vi "DAQ Judge.vi"(10 "Time and Data In":T3, 11 "Sample Settings":T1={"设备信息"={"初始索引子集"=[], "模拟信号采集通道"="Dev1", "数字-供电"="", "数字-光控"="", "光控设备"="", "光电设备分离？"=FALSE, "光谱保存路径"=path "", "环数"=0}, "测量控制"={"测头拿起"=FALSE, "起始保存"=FALSE, "测头供电"=TRUE, "测头出光"=TRUE}, "测量"={"每波长测量次数"=5, "波长"=[0, 0, 0, 0, 0, 0], "起始周期"=0, "起始测量周期"=0}, "等待"={"等待时间(s)"=0.0, "等待方式"=FALSE, "每x周期/点等待"=8, "等待时"=enum."无电无光"}, "校准"={"暗电流校准值初值"=[], "温度校准值"=[0.0, 0.0, 0.0, 0.0, 0.0, 0.0, 0.00013, 0.00013, 0.00013, 0.00013, 0.00013, 0.00013], "校准模式"=enum."逐周期"}, "图表相关"={"文件-时间"=""}, "CSM"={"CSM Name"=""}}) -> (1 "等待？":bool, 2 "Time and Data Out":T3)   [LabVIEW 2026, in "UI-无创.lvlib" / "Acquisition.lvlib"]
uses:
  Acquisition.lvlib
  Supports/Time and Data_OP.ctl
  Supports/Sample Settings.ctl
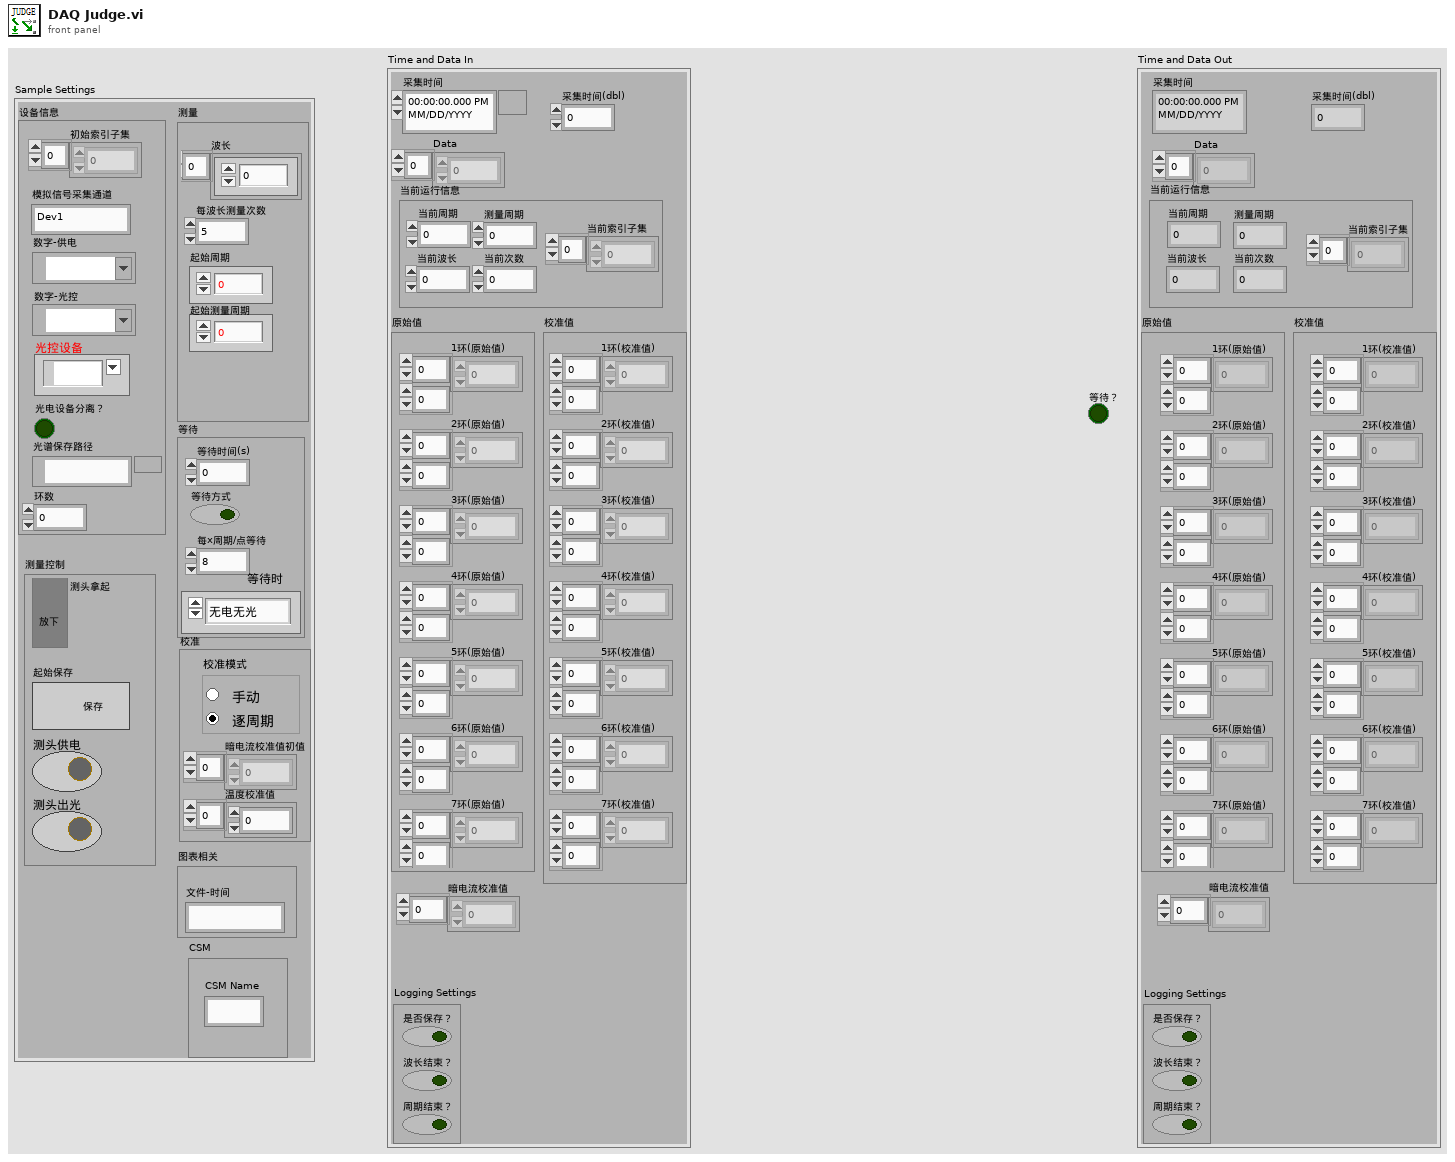
[diagram p1: front panel]
types:
  T1 = typedef "UI-无创.lvlib/Sample Settings.ctl" = cluster{"设备信息":cluster{"初始索引子集":i8[], "模拟信号采集通道":string, "数字-供电":refnum<k21>, "数字-光控":refnum<k21>, "光控设备":tag, "光电设备分离？":bool, "光谱保存路径":path, "环数":u8}, "测量控制":cluster{"测头拿起":bool, "起始保存":bool, "测头供电":bool, "测头出光":bool}, "测量":cluster{"每波长测量次数":i32, "波长":i32[], "起始周期":i32, "起始测量周期":i32}, "等待":cluster{"等待时间(s)":dbl, "等待方式":bool, "每x周期/点等待":i32, "等待时":enum16{"无电无光", "有电无光", "无电有光", "有电有光"}}, "校准":cluster{"暗电流校准值初值":dbl[], "温度校准值":dbl[], "校准模式":T2}, "图表相关":cluster{"文件-时间":string}, "CSM":cluster{"CSM Name":string}}
  T2 = typedef "UI-无创.lvlib/暗电流校准模式.ctl" = enum32{"手动", "逐周期"}
  T3 = typedef "UI-无创.lvlib/Time and Data_OP.ctl" = cluster{"采集时间":timestamp, "采集时间(dbl)":dbl, "Data":dbl[], "当前运行信息":cluster{"当前周期":i32, "当前次数":i32, "测量周期":i32, "当前索引子集":i8[], "当前波长":i32}, "暗电流校准值":dbl[], "Logging Settings":cluster{"是否保存？":bool, "波长结束？":bool, "周期结束？":bool}, "原始值":cluster{"1环(原始值)":dbl[][], "2环(原始值)":dbl[][], "3环(原始值)":dbl[][], "4环(原始值)":dbl[][], "5环(原始值)":dbl[][], "6环(原始值)":dbl[][], "7环(原始值)":dbl[][]}, "校准值":cluster{"1环(校准值)":dbl[][], "2环(校准值)":dbl[][], "3环(校准值)":dbl[][], "4环(校准值)":dbl[][], "5环(校准值)":dbl[][], "6环(校准值)":dbl[][], "7环(校准值)":dbl[][]}}
  T4 = cluster{"Time and Data In":T3, "Sample Settings":T1}
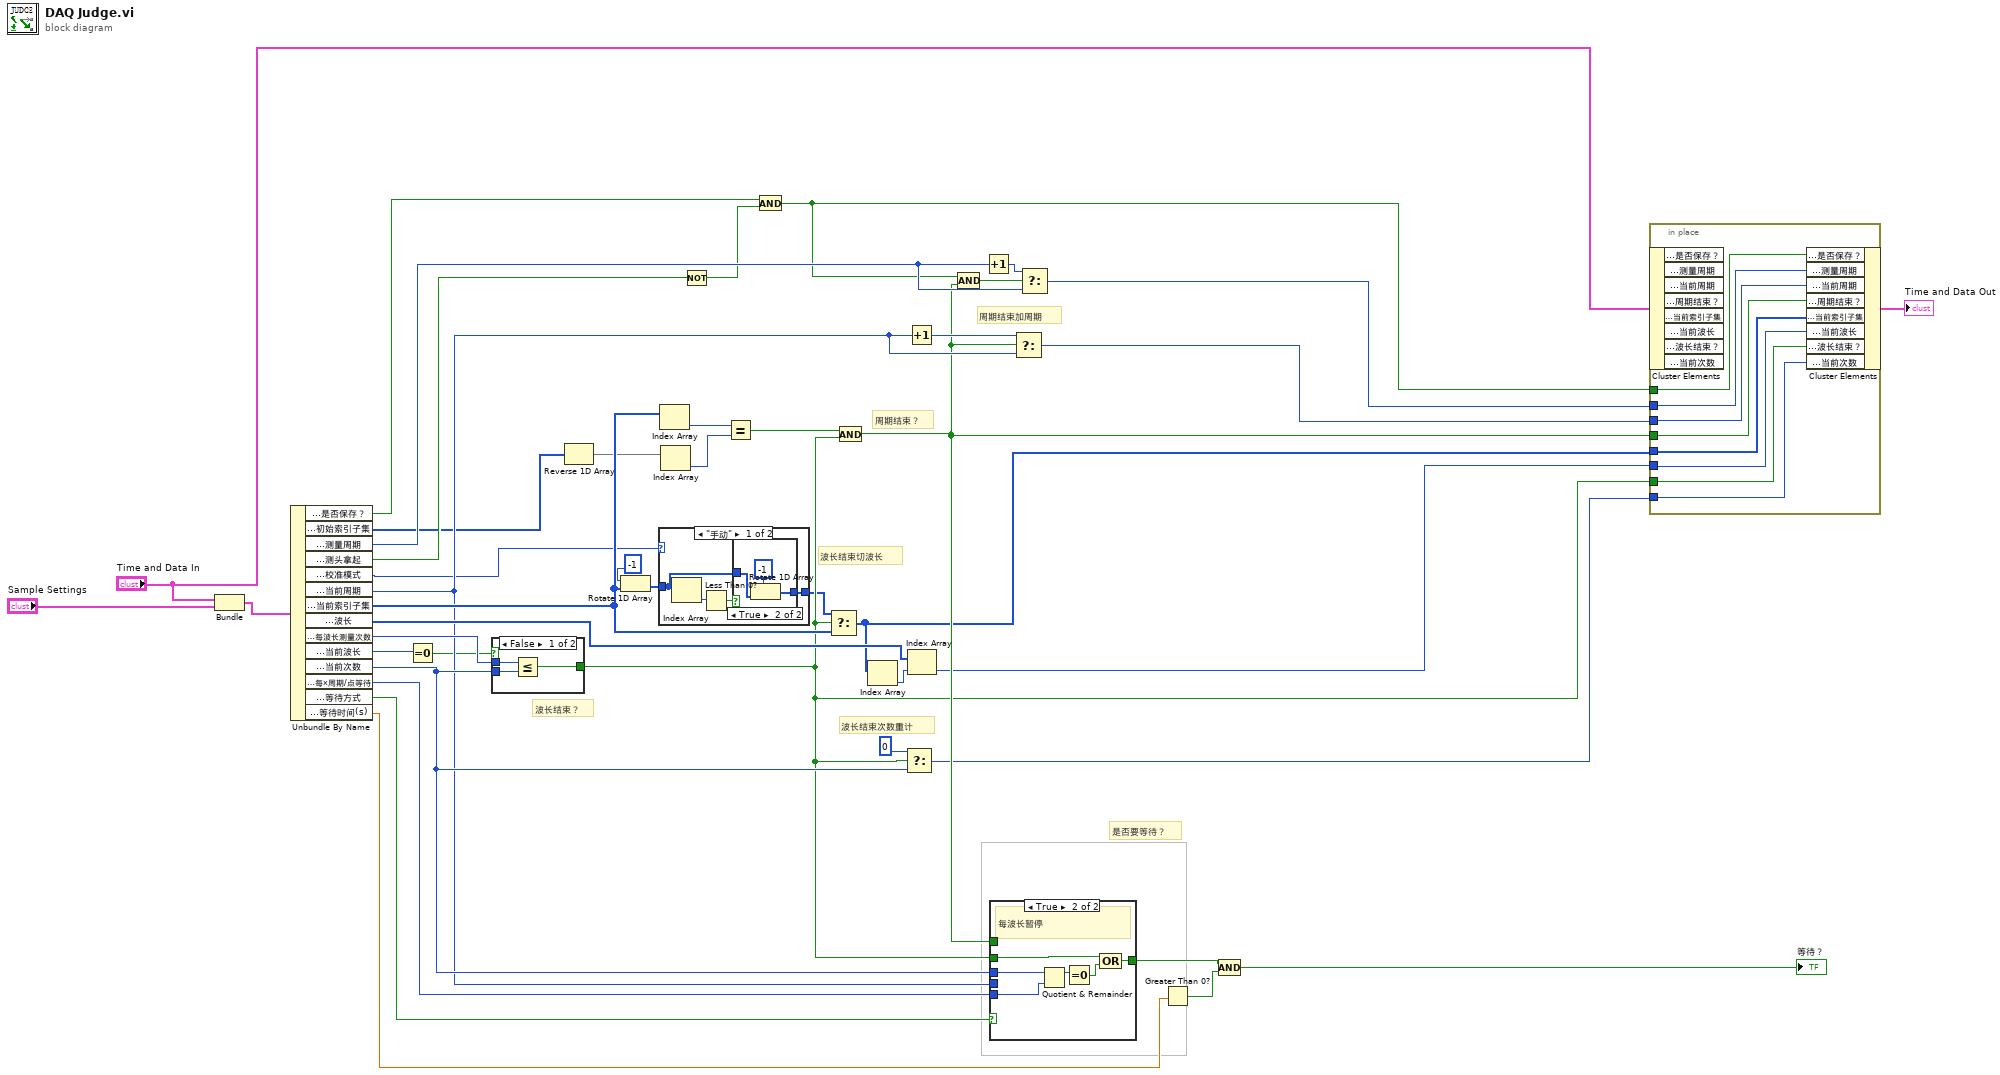
[diagram p0: block diagram]
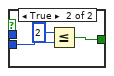
[diagram p4: hidden frame]
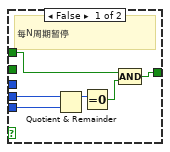
[diagram p5: hidden frame]
diagram:
  # "波长结束？"
  # "波长结束次数重计"
  # "波长结束切波长"
  # "是否要等待？"
  # "周期结束？"
  # "周期结束加周期"
  n1 = Bundle("Time and Data In"="Time and Data In", "Sample Settings"="Sample Settings") -> (w28:T4)  [unwired: 1 in]
  n2 = Unbundle By Name(w28) -> ("Time and Data In.Logging Settings.是否保存？"=w23:bool, "Sample Settings.设备信息.初始索引子集"=w7:i8[], "Time and Data In.当前运行信息.测量周期"=w30:i32, "Sample Settings.测量控制.测头拿起"=w22:bool, "Sample Settings.校准.校准模式"=w3:T2, "Time and Data In.当前运行信息.当前周期"=w33:i32, "Time and Data In.当前运行信息.当前索引子集"=w39:i8[], "Sample Settings.测量.波长"=w38:i32[], "Sample Settings.测量.每波长测量次数"=w41:i32, "Time and Data In.当前运行信息.当前波长"=w6:i32, "Time and Data In.当前运行信息.当前次数"=w34:i32, "Sample Settings.等待.每x周期/点等待"=w27:i32, "Sample Settings.等待.等待方式"=w26:bool, "Sample Settings.等待.等待时间(s)"=w20:dbl)
  n3 = Equal To 0?(x=w6) -> (x = 0?=w5:bool)
  n4 = case shown="False" w5 {
    tunnel: w41 -> [w46 _]
    tunnel: w34 -> [w45 w49]
    tunnel: [w44 w48] -> w9
    frame False {
      n5 = Less Or Equal?(x=w46, y=w45) -> (x <= y?=w44:bool)
    }
    frame True {
      n6 = Less Or Equal?(x=2, y=w49) -> (x <= y?=w48:bool)
    }
  }
  n7 = Reverse 1D Array(array=w7) -> (reversed array=w25:i8[])
  n8 = Rotate 1D Array(1:w39, 2:-1 ("n")) -> (0:w4:i8[])
  n9 = case shown="\"手动\"" w3 {
    tunnel: w4 -> [w51 w58]
    tunnel: [w50 w58] -> w2
    frame "手动" {
      n10 = Index Array(array=w51) -> (element=w53:i8)  [unwired: 1 in]
      n11 = Less Than 0?(x=w53) -> (x < 0?=w52:bool)
      n12 = case shown="True" w52 {
        tunnel: w51 -> [w54 w56]
        tunnel: [w54 w55] -> w50
        frame False {
        }
        frame True {
          n13 = Rotate 1D Array(1:w56, 2:-1 ("n")) -> (0:w55:i8[])
        }
      }
    }
    frame "逐周期", Default {
    }
  }
  n14 = Index Array(array=w39) -> (element=w35:i8)  [unwired: 1 in]
  n15 = Index Array(array=w25) -> (element=w24:i8)  [unwired: 1 in]
  n16 = Not(x=w22) -> (.not. x?=w21:bool)
  n17 = Equal?(x=w35, y=w24) -> (x = y?=w36:bool)
  n18 = Compound Arithmetic op=AND ("复合运算")(w23, w21) -> (w1:bool)
  n19 = Select(t=w2, s=w9, f=w39) -> (s? t:f=w11:i8[])
  n20 = Compound Arithmetic op=AND ("复合运算")(w36, w9) -> (w12:bool)
  n21 = Index Array(array=w11) -> (element=w40:i8)  [unwired: 1 in]
  n22 = Select(t=0, s=w9, f=w34) -> (s? t:f=w8:i32)
  n23 = Increment(x=w33) -> (x+1=w43:i32)
  n24 = Index Array(array=w38, index=w40) -> (element=w10:i32)
  n25 = Compound Arithmetic op=AND ("复合运算")(w1, w12) -> (w31:bool)
  n26 = Increment(x=w30) -> (x+1=w32:i32)
  n27 = case shown="True" w26 {
    tunnel: [w61 w70] -> w18
    tunnel: w9 -> [_ w69]
    tunnel: w12 -> [w62 _]
    tunnel: w34 -> [_ w67]
    tunnel: w33 -> [w60 _]
    tunnel: w27 -> [w59 w65]
    frame False {
      # "每N周期暂停"
      n28 = Quotient & Remainder(x=w60, y=w59) -> (x-y*floor(x/y)=w64:i32)  [unwired: 1 out]
      n29 = Equal To 0?(x=w64) -> (x = 0?=w63:bool)
      n30 = Compound Arithmetic op=AND ("复合运算")(w62, w63) -> (w61:bool)
    }
    frame True {
      # "每波长暂停"
      n31 = Quotient & Remainder(x=w67, y=w65) -> (x-y*floor(x/y)=w68:i32)  [unwired: 1 out]
      n32 = Equal To 0?(x=w68) -> (x = 0?=w66:bool)
      n33 = Compound Arithmetic op=OR ("复合运算")(w69, w66) -> (w70:bool)
    }
  }
  n34 = Select(t=w43, s=w12, f=w33) -> (s? t:f=w13:i32)
  n35 = Select(t=w32, s=w31, f=w30) -> (s? t:f=w15:i32)
  n36 = Greater Than 0?(x=w20) -> (x > 0?=w19:bool)
  n37 = Compound Arithmetic op=AND ("复合运算")(w18, w19) -> (→"等待？":bool)
  n38 = in-place {
    in-place-border: w1 -> [w78]
    in-place-border: w15 -> [w77]
    in-place-border: w13 -> [w76]
    in-place-border: w12 -> [w75]
    in-place-border: w11 -> [w74]
    in-place-border: w10 -> [w73]
    in-place-border: w9 -> [w72]
    in-place-border: w8 -> [w71]
    n39 = in-place-cluster #1("Time and Data In") -> ()  [unwired: 8 out]
    n40 = in-place-cluster #1("Logging Settings.是否保存？"=w78, "当前运行信息.测量周期"=w77, "当前运行信息.当前周期"=w76, "Logging Settings.周期结束？"=w75, "当前运行信息.当前索引子集"=w74, "当前运行信息.当前波长"=w73, "Logging Settings.波长结束？"=w72, "当前运行信息.当前次数"=w71) -> (→"Time and Data Out":T3)
  }
